vi "Spark RefNum Registry Set.vi"(8 "error in (no error)":errorcluster, 9 "Test Mode Only":bool, 10 "refnum name":string="My Motor RefNum", 11 "Spark refnum":T1) -> (0 "error out":errorcluster, 3 "Spark refnum":T1)   [LabVIEW 2023, in "REVLibDriver.lvlib"]
doc: "Sets a reference into a named registry storage. After setting a reference, you can retrieve it by name using the <B>RefNum Registry Get</B>.\nThe <B>Test Mode Only</B> parameter restricts it so Test Mode can use the reference, but other code cannot get the refnum and modify the I/O."
uses:
  <vilib>/REVLibDriver/REVLibDriver.lvlib
  <vilib>/REV Custom Controls/REVSparkRefnum.ctl
  <vilib>/Rock Robotics/WPI/Utilities/Refnum Registry Operation.ctl
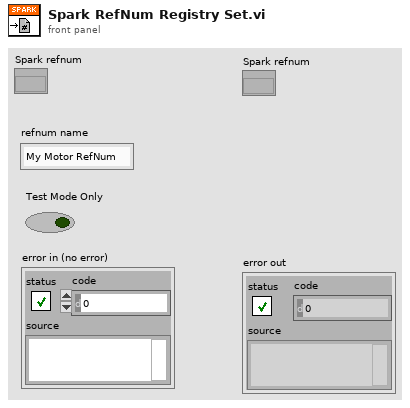
[diagram p1: front panel]
types:
  T1 = typedef "REVLibDriver.lvlib/REVSparkRefnum.ctl" = refnum<k20>
  T2 = typedef "Refnum Registry Operation.ctl" = enum16{"set", "get", "delete", "get all names", "read name"}
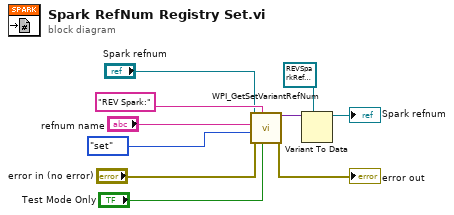
[diagram p0: block diagram]
diagram:
  n1 = call <vilib>:"WPI_GetSetVariantRefNum.vi"("Test Mode Only"="Test Mode Only", "prefix"="REV Spark:", "error in (no error)"="error in (no error)", "Operation"=Refnum_Registry_Operation."set" ("menu"), "refnum name"="refnum name", "DevRef"="Spark refnum") -> ("error out"=→"error out":errorcluster, "DevRef"=w10:variant)  [unwired: 3 in, 1 out]
  n2 = Variant To Data(type=T1 refnum ("Spark refnum"), Variant=w10) -> (data=→"Spark refnum":T1)  [unwired: 1 in, 1 out]
